vi "Consumer.vi"(8 "error in (no error)":errorcluster, 9 "Data":variant, 10 "Case ID":string, 11 "uService Template in":refnum<class "Error Manager.lvclass">) -> (0 "error out":errorcluster, 3 "uService Template out":refnum<class "Error Manager.lvclass">)   [LabVIEW 2020, in "TALOS.lvlib" / "Error Manager.lvlib" / "Error Manager.lvclass"]
uses:
  Error Manager.lvclass
  C:/LabVIEW Code/TALOS/talos/Father of all uServices/Father of all uServices/Father of all uServices.lvclass
  C:/LabVIEW Code/TALOS/builds/Actor Framework PPL/Actor Framework.lvlibp/1abvi3w/vi.lib/ActorFramework/Actor/Actor.lvclass
  Error Manager Consumer Case Selector.ctl
  Error Info.ctl
  <vilib>/Utility/error.llb/DialogType.ctl
  Guardian/Guardian Messages/Message to uService Msg/Message to uService Msg.lvclass/Message to uService Msg.ctl
  Ancestor/Ancestor/Ancestor.lvclass/Ancestor.ctl
  builds/Actor Framework PPL/Actor Framework.lvlibp/1abvi3w/vi.lib/ActorFramework/Message Enqueuer/Message Priority.ctl
  Common GUI v3/Common GUI v3/Error Listbox Msg.ctl
  Common GUI v3/Common GUI v3/Error Listbox Msg Action.ctl
  Error Manager.lvclass/Error Manager.ctl
  Father of all uServices/Father of all uServices/Father of all uServices.lvclass/Father of all uServices.ctl
  Guardian/Guardian/Requests.ctl
  Guardian/Guardian Messages/Requests from uServices Msg/Requests from uServices Msg.lvclass/Requests from uServices Msg.ctl
  FGV/Error Memory/Get All Errors Arrays.vi
  FGV/Error Memory/Error Memory Core.vi
  Guardian/Guardian Messages/Message to uService Msg/Send Message to uService.vi
  Support VIs/Generate Error.vi
  Guardian/Guardian Messages/Requests from uServices Msg/Send Requests from uServices.vi
  Support VIs/Circus Root Path.vi
  FGV/Error Memory/Error Crt Lvl checker.vi
  FGV/Error Memory/Error Memory Core.vi/40c8088d-b597-4017-91af-faa98e00292e.vi
  FGV/Error Memory/Error Memory Core.vi/d4a3ab98-063c-4e44-b43d-fbdcfe6c2be2.vi
  FGV/Error Memory/Get Error Description.vi
  Support VIs/Get PC name.vi
  Ancestor/Ancestor/Read ID.vi
  Support VIs/Get Class Name.vi
  Father of all uServices/Father of all uServices/Father of all uServices.lvclass
  Support VIs/TALOS Root path.vi
  Support VIs/Read CSV worksheet.vi
  Support VIs/Global Memory.vi
  Support VIs/Global Constants.vi
  <vilib>/Utility/error.llb/General Error Handler.vi
  builds/Actor Framework PPL/Actor Framework.lvlibp/1abvi3w/vi.lib/ActorFramework/Message Enqueuer/Enqueue.vi
  <vilib>/Utility/LVClass/Get LV Class Name.vi
  Support VIs/Error Log.vi
  <vilib>/Utility/config.llb/Open Config Data.vi
  <vilib>/Utility/config.llb/Get Section Names.vi
  <vilib>/Utility/config.llb/Get Key Names.vi
  <vilib>/Utility/config.llb/Read Key.vi
  <vilib>/Utility/config.llb/Read Key (String).vi
  <vilib>/Utility/config.llb/Close Config Data.vi
  <vilib>/Utility/error.llb/Search and Replace Pattern.vi
  <vilib>/Comparison/Equal/Equal Functor/Equal Functor.lvclass
  Guardian/Guardian Messages/Message to uService Msg/Message to uService Msg.lvclass
  Ancestor/Ancestor/Ancestor.lvclass
  Guardian/Guardian Messages/Raise Abort Msg/Raise Abort Msg.lvclass
  Guardian/Guardian Messages/Requests from uServices Msg/Requests from uServices Msg.lvclass
  TALOS.lvlib
  FGV/Error Memory/Error Memory.lvlib
  Classes/Error Filter/Error Filter.lvclass
  Common GUI v3/Common GUI v3/Common GUI v3.lvclass
  Guardian/Guardian/Guardian.lvclass
  builds/Actor Framework PPL/Actor Framework.lvlibp/1abvi3w/vi.lib/ActorFramework/Actor/Actor.lvclass
  builds/Actor Framework PPL/Actor Framework.lvlibp/1abvi3w/vi.lib/ActorFramework/Message Enqueuer/Message Enqueuer.lvclass
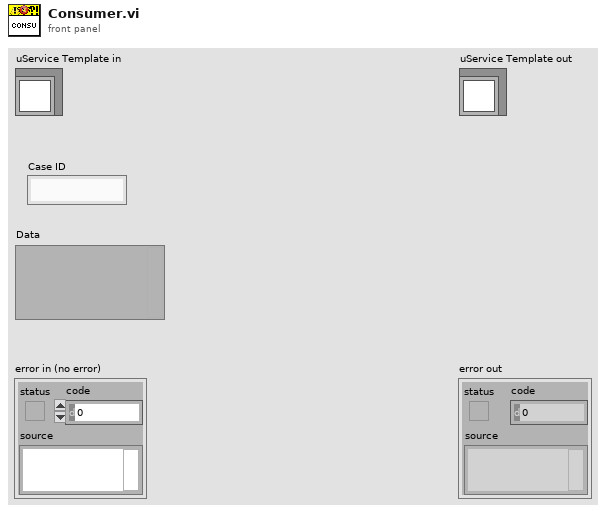
[diagram p1: front panel]
types:
  T1 = typedef "TALOS.lvlib/Error Manager.lvlib/Error Manager.lvclass/Error Manager Consumer Case Selector.ctl" = enum16{"Init", "Digest Error", "Dismiss Error", "Dismiss All", "Show Error Details", "Filter out Errors", "Clear Filters"}
  T2 = typedef "TALOS.lvlib/Error Manager.lvlib/Error Manager.lvclass/Error Info.ctl" = cluster{"error out":errorcluster, "Time Stamp":timestamp, "Machine Name":string, "GUID":string}
  T3 = typedef "Actor Framework.lvlibp/Message Enqueuer.lvclass/Message Priority.ctl" = enum16{"Low", "Normal", "High"}
  T4 = typedef "TALOS.lvlib/Common GUI v3.lvlib/Common GUI v3.lvclass/Error Listbox Msg Action.ctl" = enum16{"Add", "Remove", "Clear"}
  T5 = typedef "TALOS.lvlib/Common GUI v3.lvlib/Common GUI v3.lvclass/Error Listbox Msg.ctl" = cluster{"Action":T4, "Error Info":T2}
  T6 = typedef "TALOS.lvlib/Guardian.lvlib/Guardian.lvclass/Requests.ctl" = enum16{"Ready to Launch", "Start RUN", "Stop RUN", "Update DAQ Params", "Update Error Listbox", "Update Run Status", "Update Kasli Log", "Run Stopped with Errors", "Switch uS View"}
  T7 = typedef "DialogType.ctl" = u16
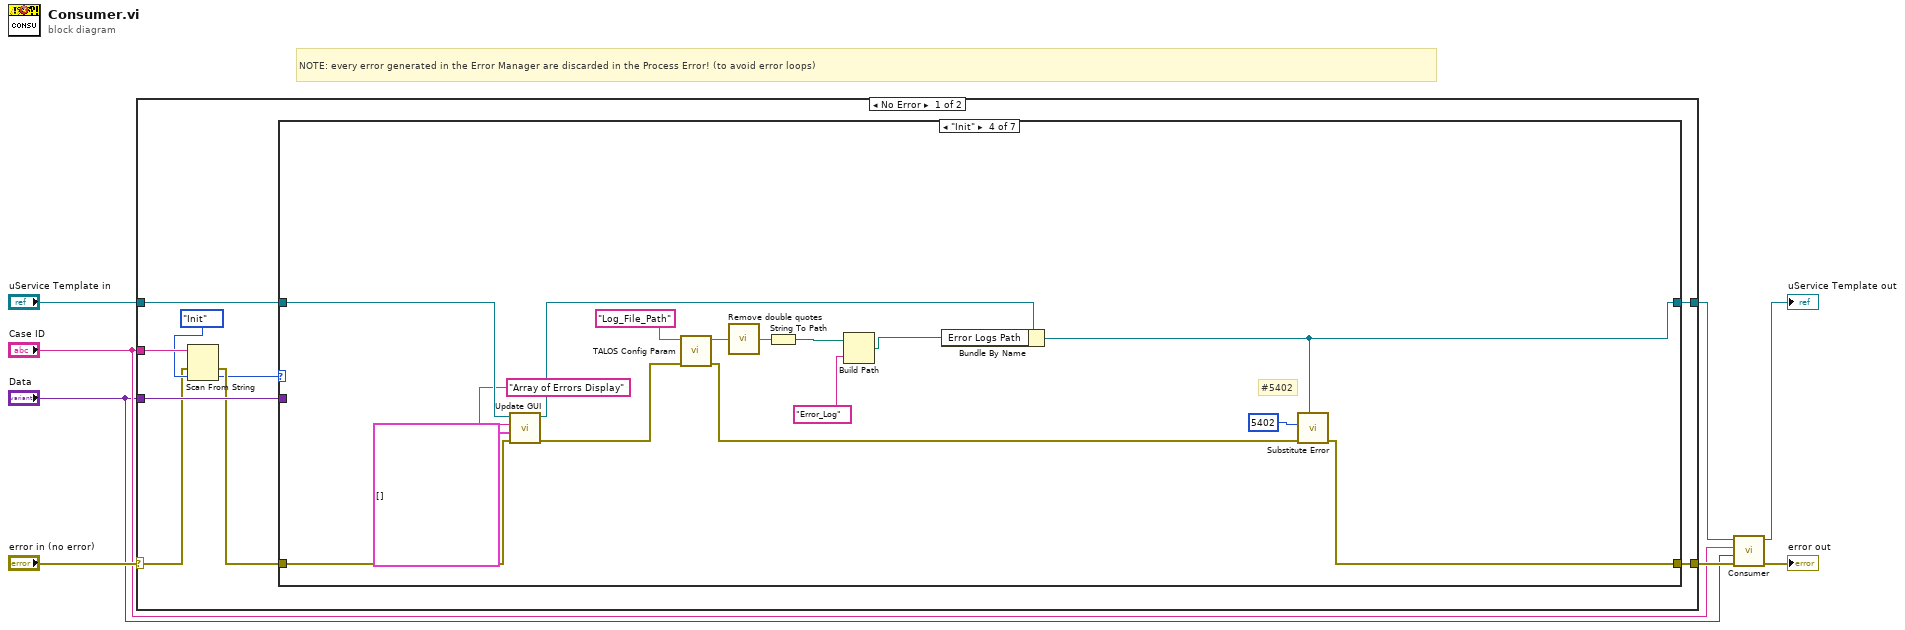
[diagram p0: block diagram]
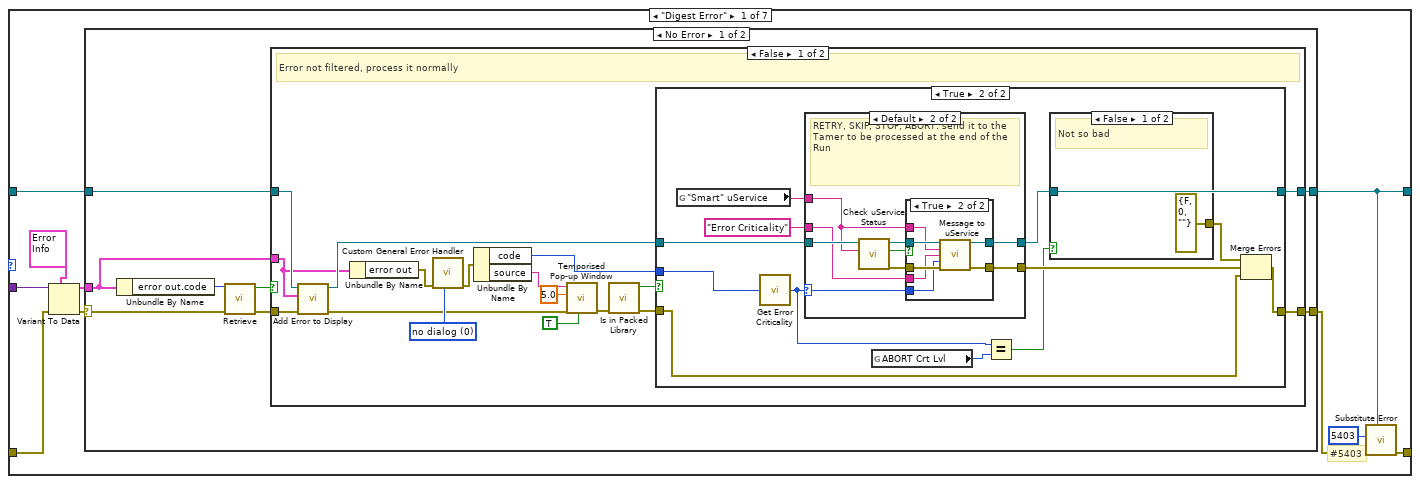
[diagram p2: hidden frame]
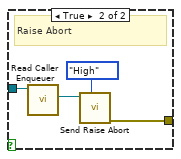
[diagram p4: hidden frame]
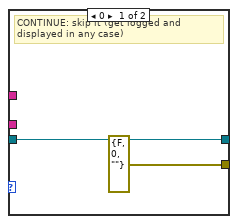
[diagram p5: hidden frame]
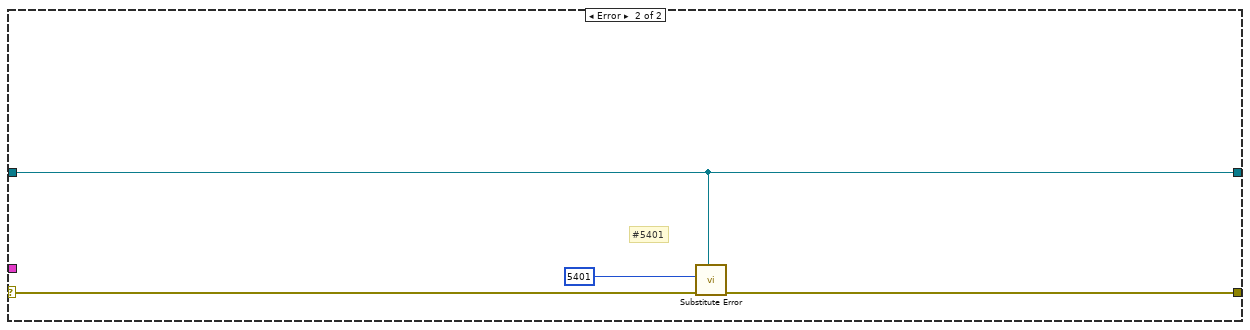
[diagram p8: hidden frame]
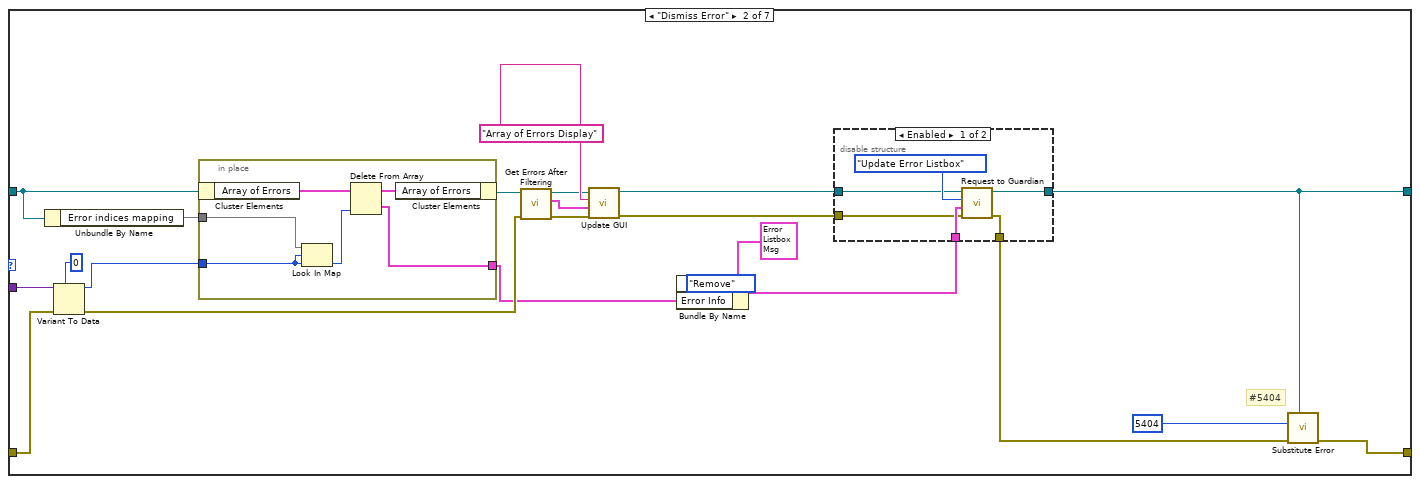
[diagram p9: hidden frame]
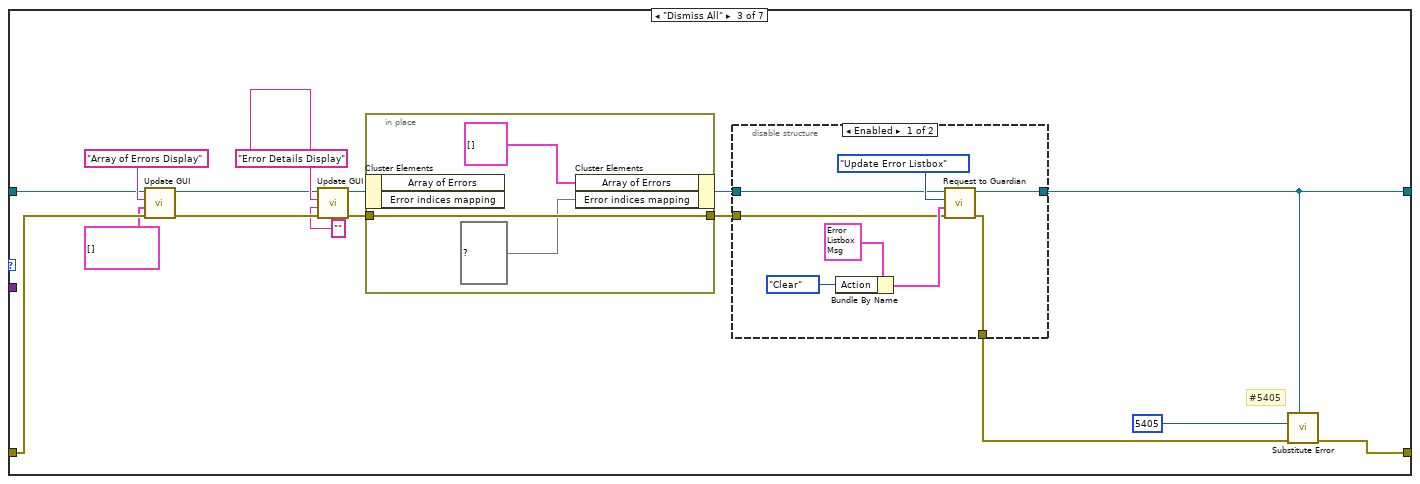
[diagram p11: hidden frame]
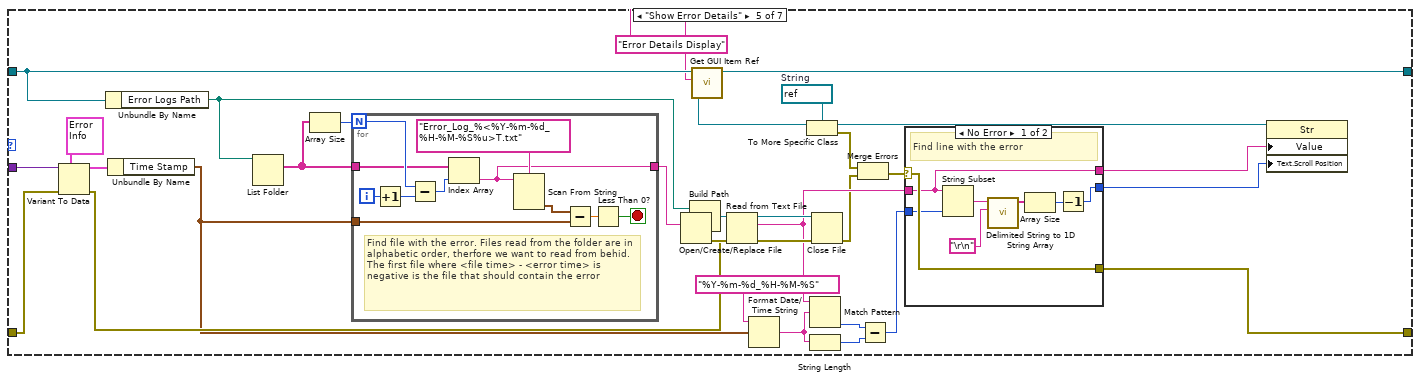
[diagram p13: hidden frame]
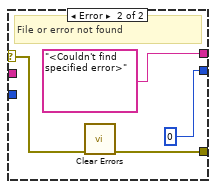
[diagram p14: hidden frame]
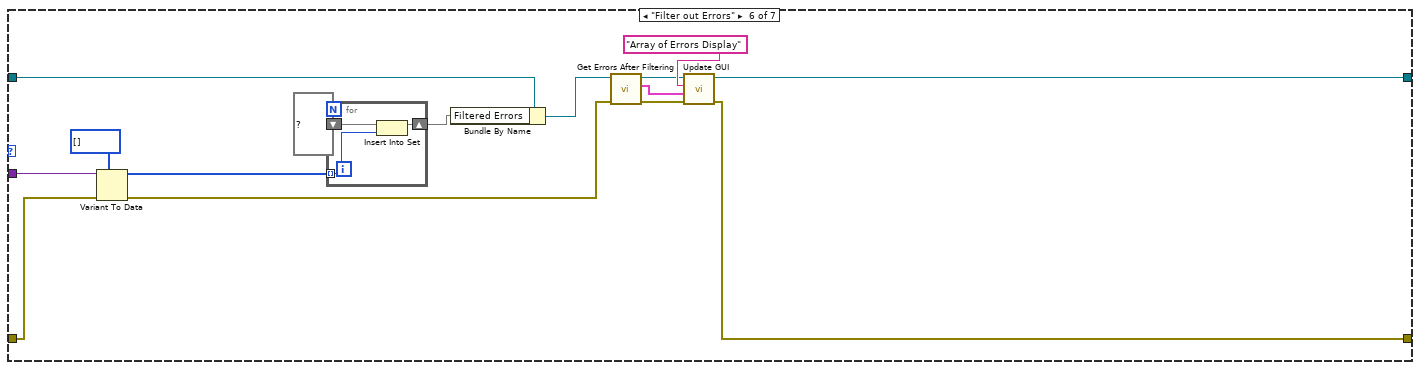
[diagram p15: hidden frame]
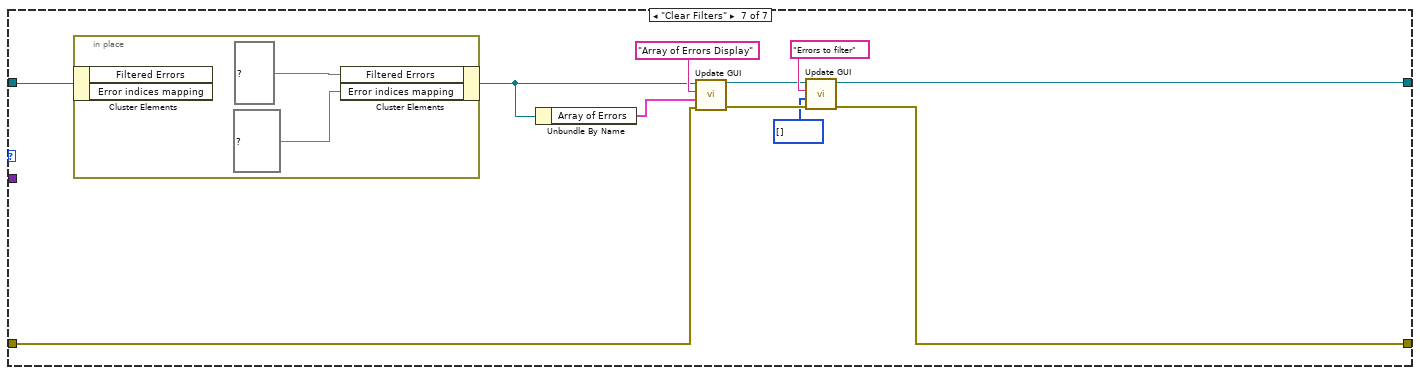
[diagram p16: hidden frame]
diagram:
  # "NOTE: every error generated in the Error Manager are discarded in the Process Error! (to avoid error loops)"
  n1 = case shown="No Error" "error in (no error)" {
    selector: "error in (no error)" -> [w12 w266]
    tunnel: [w9 w267] -> w7
    tunnel: "uService Template in" -> [w17 w267]
    tunnel: [w15 w266] -> w8
    tunnel: "Case ID" -> [w14 _]
    tunnel: "Data" -> [w16 _]
    frame No Error {
      n2 = Scan From String(input string=w14, error in=w12, default 1=Error_Manager_Consumer_Case_Selector."Init" ("ErrMgr Case Selector")) -> (error out=w11:errorcluster, output 1=w10:T1)  [unwired: 2 in, 2 out]
      n3 = case shown="\"Init\"" w10 {
        tunnel: w17 -> [w23 w101 w148 w178 w202 w246 w262]
        tunnel: w16 -> [w27 w109 _ _ w211 w249 _]
        tunnel: [w19 w113 w145 w175 w179 w238 w254] -> w15
        tunnel: w11 -> [w26 w108 w147 w176 w210 w248 w261]
        tunnel: [w18 w111 w143 w164 w201 w237 w256] -> w9
        frame "Digest Error" {
          # "#5403"
          n4 = Variant To Data(error in=w26, type=T2 {"error out"={"status"=FALSE, "code"=0, "source"=""}, "Time Stamp"=timestamp(0 s since 1904-01-01), "Machine Name"="", "GUID"=""} ("Array"), Variant=w27) -> (data=w25:T2, error out=w24:errorcluster)
          n5 = case shown="No Error" w24 {
            selector: w24 -> [w28 w96]
            tunnel: w25 -> [w31 _]
            tunnel: w23 -> [w30 w94]
            tunnel: [w34 w97] -> w20
            tunnel: [w35 w94] -> w18
            frame No Error {
              n6 = Unbundle By Name(w31) -> ("error out.code"=w29:i32)
              n7 = call "Retrieve.vi"("error in (no error)"=w28, "Error Code"=w29) -> ("error out"=w33:errorcluster, "Filter?"=w32:bool)  [unwired: 8 in]
              n8 = case shown="False" w32 {
                tunnel: w30 -> [w47 w93]
                tunnel: [w52 w93] -> w35
                tunnel: [w51 w92] -> w34
                tunnel: w33 -> [w49 w92]
                tunnel: w31 -> [w44 _]
                frame False {
                  w46 = T7 0 items=["no dialog", "OK message", "continue or stop message", "OK message + warnings", "continue/stop + warnings"] ("type of dialog (OK msg:1)")
                  # "Error not filtered, process it normally"
                  n9 = call "Add Error to Display.vi"("error in (no error)"=w49, "error to display"=w44, "Error Manager in"=w47) -> ("error out"=w45:errorcluster, "Error Manager out"=w48:refnum<class "Error Manager.lvclass">)  [unwired: 7 in]
                  n10 = Unbundle By Name(w44) -> ("error out"=w43:errorcluster)
                  n11 = call "Custom General Error Handler.vi"("type of dialog (OK msg:1)"=w46, "error in (no error)"=w43) -> ("error out"=w40:errorcluster)  [unwired: 9 in]
                  n12 = Unbundle By Name(w40) -> ("code"=w42:i32, "source"=w41:string)
                  n13 = call "Temporised Pop-up Window.vi"("error window"=TRUE, "error in (no error)"=w45, "Timeout"=5.0, "Text"=w41) -> ("error out"=w39:errorcluster)  [unwired: 7 in]
                  n14 = call "Is in Packed Library.vi"("error in (no error)"=w39) -> ("error out"=w37:errorcluster, "Is In Packed Library"=w38:bool)  [unwired: 9 in]
                  n15 = case shown="True" w38 {
                    tunnel: [w54 w56] -> w52
                    tunnel: [w53 w66] -> w51
                    tunnel: w48 -> [w54 w62]
                    tunnel: w42 -> [_ w61]
                    tunnel: w37 -> [w53 w60]
                    frame False {
                    }
                    frame True {
                      n16 = global read "Global Constants.vi" "\"Smart\" uService"() -> (w63:string)
                      n17 = call "Get Error Criticality.vi"("Error Code in"=w61) -> ("Error Criticality"=w58:u8)  [unwired: 4 in]
                      n18 = case shown="Default" w58 {
                        selector: w58 -> [_ w76]
                        tunnel: w62 -> [w73 w78]
                        tunnel: [w73 w81] -> w56
                        tunnel: [errorcluster {"status"=FALSE, "code"=0, "source"=""} ("error out") w82] -> w65
                        tunnel: "Error Criticality" ("Message") -> [_ w77]
                        tunnel: w63 -> [_ w75]
                        frame 0 {
                          # "CONTINUE: skip it (get logged and displayed in any case)"
                        }
                        frame Default {
                          # "RETRY, SKIP, STOP, ABORT: send it to the Tamer to be processed at the end of the Run"
                          n19 = call-dynamic "Check uService Status.vi"("uService ID"=w75, "Father of all uServices in"=w78) -> ("error out"=w79:errorcluster, "Online?"=w74:bool, "Father of all uServices out"=w80:refnum<class "Error Manager.lvclass">)  [unwired: 6 in, 1 out]
                          n20 = case shown="True" w74 {
                            tunnel: [w83 w91] -> w82
                            tunnel: [w84 w90] -> w81
                            tunnel: w80 -> [w84 w89]
                            tunnel: w79 -> [w83 w88]
                            tunnel: w77 -> [_ w87]
                            tunnel: w76 -> [_ w86]
                            tunnel: w75 -> [_ w85]
                            frame False {
                            }
                            frame True {
                              n21 = call "Message to uService.vi"("Father of all uServices in"=w89, "uService ID"=w85, "Message"=w87, "Data"=w86, "error in (no error)"=w88) -> ("Father of all uServices out"=w90:refnum<class "Error Manager.lvclass">, "error out"=w91:errorcluster)  [unwired: 9 in]
                            }
                          }
                        }
                      }
                      n22 = global read "Global Constants.vi" "ABORT Crt Lvl"() -> (w59:u8)
                      n23 = Equal?(x=w58, y=w59) -> (x = y?=w57:bool)
                      n24 = case shown="False" w57 {
                        tunnel: w56 -> [_ w71]
                        tunnel: [errorcluster {"status"=FALSE, "code"=0, "source"=""} ("error out") w68] -> w55
                        frame False {
                          # "Not so bad"
                        }
                        frame True {
                          # "Raise Abort"
                          n25 = call "Read Caller Enqueuer.vi"("Actor"=w71) -> ("Caller Enqueuer"=w70:refnum<class "Message Enqueuer.lvclass">)  [unwired: 10 in]
                          n26 = call "Send Raise Abort.vi"("Message Priority (Normal)"=Message_Priority."High", "Message Enqueuer"=w70) -> ("error out"=w68:errorcluster)  [unwired: 8 in, 1 out]
                        }
                      }
                      n27 = Merge Errors(w55, w65, w60) -> (w66:errorcluster)
                    }
                  }
                }
                frame True {
                  # "Error filtered, skip it"
                }
              }
            }
            frame Error {
              # "#5401"
              n28 = call "Substitute Error.vi"("LabVIEW Object"=w94, "error in (no error)"=w96, "Error Code"=5401) -> ("error out"=w97:errorcluster)  [unwired: 8 in]
            }
          }
          n29 = call "Substitute Error.vi"("LabVIEW Object"=w18, "error in (no error)"=w20, "Error Code"=5403) -> ("error out"=w19:errorcluster)  [unwired: 8 in]
        }
        frame "Dismiss Error" {
          # "#5404"
          n30 = Unbundle By Name(w101) -> ("Error indices mapping"=w100:map{i32, i32})
          n31 = Variant To Data(error in=w108, type=0 ("Select Error"), Variant=w109) -> (data=w99:i32, error out=w119:errorcluster)
          n32 = in-place {
            in-place-border: w100 -> [w122]
            in-place-border: w99 -> [w121]
            in-place-border: [w120] -> w98
            n33 = in-place-cluster #1(w101) -> ("Array of Errors"=w125:T2[])
            n34 = Look In Map(map=w122, key=w121, default value=w121) -> (value=w123:i32)  [unwired: 1 out]
            n35 = Delete From Array(array=w125, index=w123) -> (deleted portion=w120:T2, array with subset deleted=w124:T2[])  [unwired: 1 in]
            n36 = in-place-cluster #1("Array of Errors"=w124) -> (w107:refnum<class "Error Manager.lvclass">)
          }
          n37 = call-dynamic "Get Errors After Filtering.vi"("error in (no error)"=w119, "Error Manager in"=w107) -> ("error out"=w104:errorcluster, "Array of Errors"=w105:T2[], "Error Manager out"=w106:refnum<class "Error Manager.lvclass">)  [unwired: 7 in]
          n38 = call "Update GUI.vi"("error in (no error)"=w104, "Data"=w105, "GUI Item Name"="Array of Errors Display" ("FP Item Name"), "uService Template in"=w106) -> ("error out"=w102:errorcluster, "uService Template out"=w103:refnum<class "Error Manager.lvclass">)  [unwired: 6 in]
          n39 = Bundle By Name(cluster=T5 {"Action"=enum."Add", "Error Info"={"error out"={"status"=FALSE, "code"=0, "source"=""}, "Time Stamp"=timestamp(0 s since 1904-01-01), "Machine Name"="", "GUID"=""}} ("Error Listbox Msg"), "Action"=Error_Listbox_Msg_Action."Remove", "Error Info"=w98) -> (w115:T5)
          n40 = disable-structure shown="Enabled" {
            disable-tunnel: w115 -> [w131 _]
            disable-tunnel: [w129 w132] -> w112
            disable-tunnel: [w128 w133] -> w111
            disable-tunnel: w102 -> [w127 w132]
            disable-tunnel: w103 -> [w126 w133]
            frame Enabled {
              n41 = call "Request to Guardian.vi"("error in (no error)"=w127, "Data"=w131, "Requests"=Requests."Update Error Listbox", "Father of all uServices in"=w126) -> ("error out"=w129:errorcluster, "Father of all uServices out"=w128:refnum<class "Error Manager.lvclass">)  [unwired: 6 in]
            }
            frame Disabled {
            }
          }
          n42 = call "Substitute Error.vi"("LabVIEW Object"=w111, "error in (no error)"=w112, "Error Code"=5404) -> ("error out"=w113:errorcluster)  [unwired: 8 in]
        }
        frame "Dismiss All" {
          # "#5405"
          n43 = call "Update GUI.vi"("error in (no error)"=w147, "Data"=T2[] [] ("error constant"), "GUI Item Name"="Array of Errors Display" ("FP Item Name"), "uService Template in"=w148) -> ("error out"=w139:errorcluster, "uService Template out"=w140:refnum<class "Error Manager.lvclass">)  [unwired: 6 in]
          n44 = call "Update GUI.vi"("error in (no error)"=w139, "Data"="", "GUI Item Name"="Error Details Display", "uService Template in"=w140) -> ("error out"=w136:errorcluster, "uService Template out"=w137:refnum<class "Error Manager.lvclass">)  [unwired: 6 in]
          n45 = in-place {
            in-place-border: w136 -> [w152]
            in-place-border: [w152] -> w134
            n46 = in-place-cluster #2(w137) -> ()  [unwired: 2 out]
            n47 = in-place-cluster #2("Array of Errors"=T2[] [], "Error indices mapping"=map{i32, i32} {}) -> (w135:refnum<class "Error Manager.lvclass">)
          }
          n48 = disable-structure shown="Enabled" {
            disable-tunnel: [w156 w161] -> w144
            disable-tunnel: [w155 w162] -> w143
            disable-tunnel: w135 -> [w154 w162]
            disable-tunnel: w134 -> [w153 w161]
            frame Enabled {
              n49 = Bundle By Name(cluster=T5 {"Action"=enum."Add", "Error Info"={"error out"={"status"=FALSE, "code"=0, "source"=""}, "Time Stamp"=timestamp(0 s since 1904-01-01), "Machine Name"="", "GUID"=""}} ("Error Listbox Msg"), "Action"=Error_Listbox_Msg_Action."Clear") -> (w158:T5)
              n50 = call "Request to Guardian.vi"("error in (no error)"=w153, "Data"=w158, "Requests"=Requests."Update Error Listbox", "Father of all uServices in"=w154) -> ("error out"=w156:errorcluster, "Father of all uServices out"=w155:refnum<class "Error Manager.lvclass">)  [unwired: 6 in]
            }
            frame Disabled {
            }
          }
          n51 = call "Substitute Error.vi"("LabVIEW Object"=w143, "error in (no error)"=w144, "Error Code"=5405) -> ("error out"=w145:errorcluster)  [unwired: 8 in]
        }
        frame "Init" {
          # "#5402"
          n52 = call "Update GUI.vi"("error in (no error)"=w176, "Data"=T2[] [] ("Array"), "GUI Item Name"="Array of Errors Display" ("FP Item Name"), "uService Template in"=w178) -> ("error out"=w167:errorcluster, "uService Template out"=w165:refnum<class "Error Manager.lvclass">)  [unwired: 6 in]
          n53 = call "TALOS Config Param.vi"("error in (no error)"=w167, "Parameter Name"="Log_File_Path") -> ("error out"=w166:errorcluster, "Output"=w172:string)  [unwired: 8 in]
          n54 = call "Remove double quotes.vi"("Input string"=w172) -> ("Output string"=w171:string)  [unwired: 4 in]
          n55 = String To Path(string=w171) -> (path=w170:path)
          n56 = Build Path(base path=w170, name or relative path="Error_Log") -> (appended path=w163:path)
          n57 = Bundle By Name(cluster=w165, "Error Logs Path"=w163) -> (w164:refnum<class "Error Manager.lvclass">)
          n58 = call "Substitute Error.vi"("LabVIEW Object"=w164, "error in (no error)"=w166, "Error Code"=5402) -> ("error out"=w175:errorcluster)  [unwired: 8 in]
        }
        frame "Show Error Details" {
          w192 = refnum<vi> refnum  # String
          n59 = Variant To Data(error in=w210, type=T2 {"error out"={"status"=FALSE, "code"=0, "source"=""}, "Time Stamp"=timestamp(0 s since 1904-01-01), "Machine Name"="", "GUID"=""} ("Error Info"), Variant=w211) -> (data=w208:T2, error out=w197:errorcluster)
          n60 = Unbundle By Name(w202) -> ("Error Logs Path"=w207:path)
          n61 = Unbundle By Name(w208) -> ("Time Stamp"=w191:timestamp)
          n62 = List Folder(path=w207) -> (filenames=w205:string[])  [unwired: 3 in, 3 out]
          n63 = Array Size(array=w205) -> (size(s)=w206:i32)
          n64 = for {
            N: w206 -> [w233]
            tunnel: w205 -> [w231]
            tunnel: w191 -> [w227]
            tunnel: [w224] -> w204
            i -> [w234]
            stop <- w225 stop-if-true
            # "Find file with the error. Files read from the folder are in alphabetic order, therfore we want to read from behid. The first file where <file time> - <error time> is negative is the file that should contain the error"
            n65 = Increment(x=w234) -> (x+1=w232:i32)
            n66 = Subtract(x=w233, y=w232) -> (x-y=w230:i32)
            n67 = Index Array(array=w231, index=w230) -> (element=w224:string)
            n68 = Scan From String(format string="Error_Log_%<%Y-%m-%d_%H-%M-%S%u>T.txt", input string=w224) -> (output 1=w228:timestamp)  [unwired: 3 in, 3 out]
            n69 = Subtract(x=w228, y=w227) -> (x-y=w226:dbl)
            n70 = Less Than 0?(x=w226) -> (x < 0?=w225:bool)
          }
          n71 = Build Path(base path=w207, name or relative path=w204) -> (appended path=w203:path)
          n72 = Open/Create/Replace File(file path (use dialog)=w203, error in=w197) -> (refnum out=w199:refnum<file>, error out=w198:errorcluster)  [unwired: 4 in, 1 out]
          n73 = call "Get GUI Item Ref.vi"("FP Item Name"="Error Details Display", "uService Template in"=w202) -> ("Ctl Refnum"=w194:refnum<vi>, "uService Template out"=w201:refnum<class "Error Manager.lvclass">)  [unwired: 7 in, 1 out]
          n74 = Read from Text File(file (use dialog)=w199, error in=w198) -> (refnum out=w195:refnum<file>, text=w186:string, error out=w196:errorcluster)  [unwired: 2 in, 1 out]
          n75 = Format Date/Time String(time format string (%c)="%Y-%m-%d_%H-%M-%S", seconds (now)=w191) -> (date/time string=w188:string)  [unwired: 1 in]
          n76 = To More Specific Class(target class=w192, reference=w194) -> (specific class reference=w193:refnum<vi>, error out=w183:errorcluster)  [unwired: 1 in]
          n77 = Match Pattern(string=w186, regular expression=w188) -> (offset past match=w187:i32)  [unwired: 1 in, 3 out]
          n78 = String Length(string=w188) -> (length=w189:i32)
          n79 = Close File(refnum=w195, error in=w196) -> (error out=w182:errorcluster)  [unwired: 1 out]
          n80 = Merge Errors(w183, w182) -> (w181:errorcluster)
          n81 = Subtract(x=w187, y=w189) -> (x-y=w184:i32)
          n82 = case shown="No Error" w181 {
            selector: w181 -> [w219 w221]
            tunnel: w186 -> [w212 _]
            tunnel: [w214 0] -> w185
            tunnel: w184 -> [w213 _]
            tunnel: [w212 "<Couldn't find specified error>"] -> w180
            tunnel: [w219 w220] -> w179
            frame No Error {
              # "Find line with the error"
              n83 = String Subset(string=w212, length (rest)=w213) -> (substring=w215:string)  [unwired: 1 in]
              n84 = call <vilib>:"Delimited String to 1D String Array.vi"("delimiter"="\r\n", "delimited string"=w215) -> ("string array"=w217:string[])  [unwired: 9 in]
              n85 = Array Size(array=w217) -> (size(s)=w216:i32)
              n86 = Decrement(x=w216) -> (x-1=w214:i32)
            }
            frame Error {
              # "File or error not found"
              n87 = call <vilib>:"Clear Errors.vi"("error in (no error)"=w221) -> ("error out"=w220:errorcluster)  [unwired: 5 in, 1 out]
            }
          }
          n88 = property class="Str"(reference=w193, "Value"=w180, "Text.Scroll Position"=w185) -> ()  [unwired: 1 in, 2 out]
        }
        frame "Filter out Errors" {
          n89 = Variant To Data(error in=w248, type=i32[] [], Variant=w249) -> (data=w245:i32[], error out=w243:errorcluster)
          n90 = for {
            tunnel: w245 -> [w251] mode=indexing
            shift-right: [w250] -> w235
            shift-left: set{i32} {} ("Filtered Errors") -> [w252]
            n91 = Insert Into Set(10:w251, 11:w252) -> (3:w250:set{i32})  [unwired: 1 out]
          }
          n92 = Bundle By Name(cluster=w246, "Filtered Errors"=w235) -> (w244:refnum<class "Error Manager.lvclass">)
          n93 = call-dynamic "Get Errors After Filtering.vi"("error in (no error)"=w243, "Error Manager in"=w244) -> ("error out"=w240:errorcluster, "Array of Errors"=w239:T2[], "Error Manager out"=w241:refnum<class "Error Manager.lvclass">)  [unwired: 7 in]
          n94 = call "Update GUI.vi"("error in (no error)"=w240, "Data"=w239, "GUI Item Name"="Array of Errors Display" ("FP Item Name"), "uService Template in"=w241) -> ("error out"=w238:errorcluster, "uService Template out"=w237:refnum<class "Error Manager.lvclass">)  [unwired: 6 in]
        }
        frame "Clear Filters" {
          n95 = in-place {
            n96 = in-place-cluster #3(w262) -> ()  [unwired: 2 out]
            n97 = in-place-cluster #3("Filtered Errors"=set{i32} {}, "Error indices mapping"=map{i32, i32} {}) -> (w260:refnum<class "Error Manager.lvclass">)
          }
          n98 = Unbundle By Name(w260) -> ("Array of Errors"=w259:T2[])
          n99 = call "Update GUI.vi"("error in (no error)"=w261, "Data"=w259, "GUI Item Name"="Array of Errors Display" ("FP Item Name"), "uService Template in"=w260) -> ("error out"=w255:errorcluster, "uService Template out"=w257:refnum<class "Error Manager.lvclass">)  [unwired: 6 in]
          n100 = call "Update GUI.vi"("error in (no error)"=w255, "Data"=i32[] [], "GUI Item Name"="Errors to filter" ("FP Item Name"), "uService Template in"=w257) -> ("error out"=w254:errorcluster, "uService Template out"=w256:refnum<class "Error Manager.lvclass">)  [unwired: 6 in]
        }
      }
    }
    frame Error {
    }
  }
  n101 = call-parent "Consumer.vi"("error in (no error)"=w8, "Data"="Data", "Case ID"="Case ID", "uService Template in"=w7) -> ("error out"=→"error out":errorcluster, "uService Template out"=→"uService Template out":refnum<class "Error Manager.lvclass">)  [unwired: 6 in]
